vi "MedianFilter_Execute.vi"(9 "Enable":bool=TRUE, 10 "Samples":i32, 11 "Input Value":dbl) -> (1 "MedianValue":dbl, 3 "Out MEDIAN_FILTER":T1 {"ValueBuffer" format="%13.5g"})   [LabVIEW 2019, in "Trajectory_Library.lvlib"]
doc: "Convience, single call, LabVIEW function. Creates and calculates the moving-window median for the next value of the input stream.\nThe optional enable parameter bypasses the filter calculation when \"enabled\" is false. When enabled is \"false\" the internal buffer is continually filled with the current input value.\n\nThis implements a moving-window median filter. Useful for reducing measurement noise, especially with processes that generate occasional, extreme outliers (such as values from vision processing, LIDAR, or ultrasonic sensors).\n\nInputs:\n - Input Value -- The next input value. \n - samples -- The number of samples in the moving window.\n - enable -- Perform the filter calcuation when True. When False, output the input value unchanged. (Default=True)\n\nOutputs:\n - Out Median Filter -- Updated median filter data structure\n - Median Value -- The median of the moving window, updated to include the next value.."
uses:
  Trajectory_Library.lvlib
  TypeDef/MEDIAN_FILTER.ctl
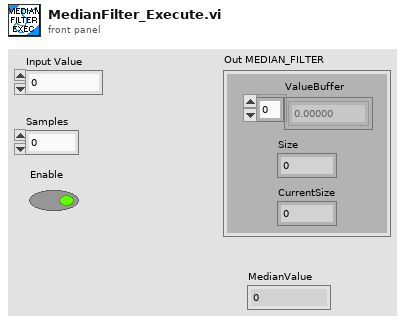
[diagram p1: front panel]
types:
  T1 = typedef "Trajectory_Library.lvlib/MEDIAN_FILTER.ctl" = cluster{"ValueBuffer":dbl[], "Size":i32, "CurrentSize":i32}
  T2 = typedef "WPILib_Math.lvlib/MEDIAN_FILTER.ctl" = cluster{"ValueBuffer":dbl[], "Size":i32, "CurrentSize":i32}
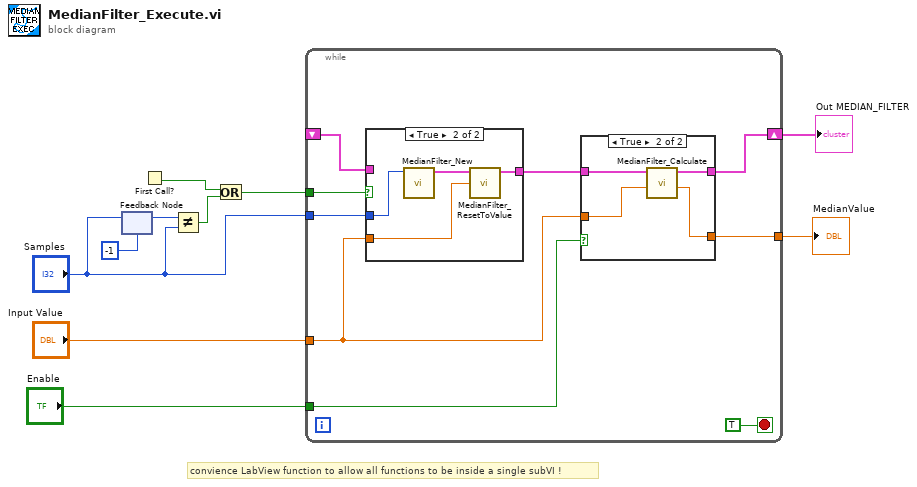
[diagram p0: block diagram]
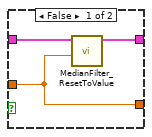
[diagram p2: hidden frame]
diagram:
  # "convience LabView function to allow all functions to be inside a single subVI !"
  n1 = feedback-in #1("Samples") -> ()
  n2 = feedback #1(-1 ("Samples")) -> (w5:i32)
  n3 = First Call?() -> (First Call?: T/F=w2:bool)
  n4 = Not Equal?(x=w5, y="Samples") -> (x != y?=w6:bool)
  n5 = Or(x=w2, y=w6) -> (x .or. y?=w7:bool)
  n6 = while {
    tunnel: "Enable" -> [w19]
    tunnel: w7 -> [w16]
    tunnel: "Samples" -> [w15]
    tunnel: "Input Value" -> [w13]
    tunnel: [w18] -> w9
    shift-right: [w17] -> w8
    shift-left: _ -> [w12]
    stop <- TRUE stop-if-true
    n7 = case shown="True" w16 {
      tunnel: w12 -> [w27 _]
      tunnel: w15 -> [_ w30]
      tunnel: w13 -> [_ w29]
      tunnel: [w27 w28] -> w14
      frame False {
      }
      frame True {
        n8 = call "MedianFilter_New.vi"("Samples"=w30) -> ("MEDIAN_FILTER"=w31:T2)  [unwired: 10 in]
        n9 = call "MedianFilter_ResetToValue.vi"("Value"=w29, "In MEDIAN_FILTER"=w31) -> ("Out MEDIAN_FILTER"=w28:T2)  [unwired: 9 in]
      }
    }
    n10 = case shown="True" w19 {
      tunnel: w14 -> [w22 w26]
      tunnel: [w21 w25] -> w17
      tunnel: w13 -> [w20 w24]
      tunnel: [w20 w23] -> w18
      frame False {
        n11 = call "MedianFilter_ResetToValue.vi"("Value"=w20, "In MEDIAN_FILTER"=w22) -> ("Out MEDIAN_FILTER"=w21:T2)  [unwired: 9 in]
      }
      frame True {
        n12 = call "MedianFilter_Calculate.vi"("Input Value"=w24, "In MEDIAN_FILTER"=w26) -> ("MedianValue"=w23:dbl, "Out MEDIAN_FILTER"=w25:T2)  [unwired: 8 in]
      }
    }
  }
  "Out MEDIAN_FILTER" <- w8
  "MedianValue" <- w9
